vi "PathPlanner_PathPoint_Equals.vi"(9 "Other PathPlannerPoint":T1={"Position"={"X"=0.0, "Y"=0.0}, "DistAlongPath"=0.0, "MaxV"=9e+300, "Constraints"={"MaxVelocityMps;"=0.0, "MaxAccelerationMpsSq;"=0.0, "MaxAngularVelRadPsEc;"=0.0, "MaxAngularAccRadPSecSq"=0.0, "Exists"=FALSE, "Unlimited"=FALSE, "NominalVoltageVolts"=0.0}, "RotationTarget"={"rotation"={"VALUE"=0.0, "COS"=1.0, "SIN"=0.0}, "position"=1.0, "Exists"=FALSE}, "WaypointRelativePos"=0.0} {"RotationTarget"."rotation"."SIN" format="%13.4f"; "RotationTarget"."rotation"."COS" format="%13.4f"; "RotationTarget"."rotation"."VALUE" format="%13.4f"; "Position"."Y" format="%14.3f"; "Position"."X" format="%14.3f"}, 11 "PathPlannerPoint":T1={"Position"={"X"=0.0, "Y"=0.0}, "DistAlongPath"=0.0, "MaxV"=9e+300, "Constraints"={"MaxVelocityMps;"=0.0, "MaxAccelerationMpsSq;"=0.0, "MaxAngularVelRadPsEc;"=0.0, "MaxAngularAccRadPSecSq"=0.0, "Exists"=FALSE, "Unlimited"=FALSE, "NominalVoltageVolts"=0.0}, "RotationTarget"={"rotation"={"VALUE"=0.0, "COS"=1.0, "SIN"=0.0}, "position"=1.0, "Exists"=FALSE}, "WaypointRelativePos"=0.0} {"RotationTarget"."rotation"."SIN" format="%13.4f"; "RotationTarget"."rotation"."COS" format="%13.4f"; "RotationTarget"."rotation"."VALUE" format="%13.4f"; "Position"."Y" format="%14.3f"; "Position"."X" format="%14.3f"}) -> (3 "Equal":bool)   [LabVIEW 2019, in "PathPlanner24.lvlib"]
doc: "Determines if two Path Point definitions are equal\n\nInputs:\n -- PathPoint - cluster - point definition\n -- Other PathPoint - cluster - point definition\n\nOutputs:\n -- Equal - boolean - TRUE if both definitions are the same."
uses:
  PathPlanner24.lvlib
  <vilib>/Rock Robotics/WPI/ThirdParty/JAS_Junk/TrajLib/Trajectory_Library.lvlib
  <vilib>/Rock Robotics/WPI/ThirdParty/JAS_Junk/TrajLib/TypeDef/ROTATION2D.ctl
  <vilib>/Rock Robotics/WPI/ThirdParty/JAS_Junk/TrajLib/TypeDef/TRANSLATION2D.ctl
  TypeDef/PathPlannerPathConstraints.ctl
  TypeDef/PathPlannerPathPoint.ctl
  TypeDef/PathPlannerRotationTarget.ctl
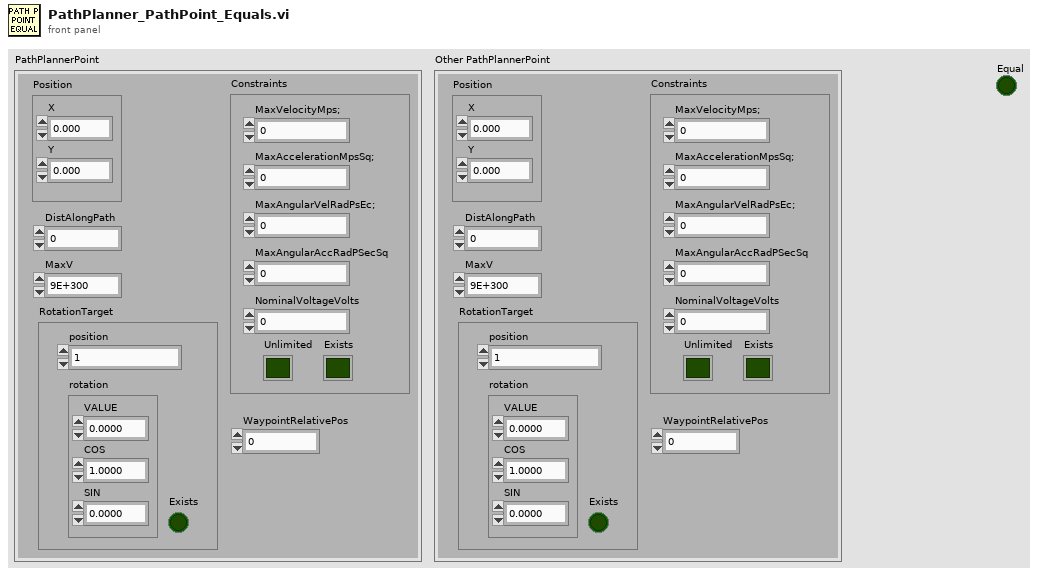
[diagram p1: front panel]
types:
  T1 = typedef "PathPlanner24.lvlib/PathPlannerPathPoint.ctl" = cluster{"Position":T2, "DistAlongPath":dbl, "MaxV":dbl, "Constraints":T3, "RotationTarget":T4, "WaypointRelativePos":dbl}
  T2 = typedef "Trajectory_Library.lvlib/TRANSLATION2D.ctl" = cluster{"X":dbl, "Y":dbl}
  T3 = typedef "PathPlanner24.lvlib/PathPlannerPathConstraints.ctl" = cluster{"MaxVelocityMps;":dbl, "MaxAccelerationMpsSq;":dbl, "MaxAngularVelRadPsEc;":dbl, "MaxAngularAccRadPSecSq":dbl, "Exists":bool, "Unlimited":bool, "NominalVoltageVolts":dbl}
  T4 = typedef "PathPlanner24.lvlib/PathPlannerRotationTarget.ctl" = cluster{"rotation":T5, "position":dbl, "Exists":bool}
  T5 = typedef "Trajectory_Library.lvlib/ROTATION2D.ctl" = cluster{"VALUE":dbl, "COS":dbl, "SIN":dbl}
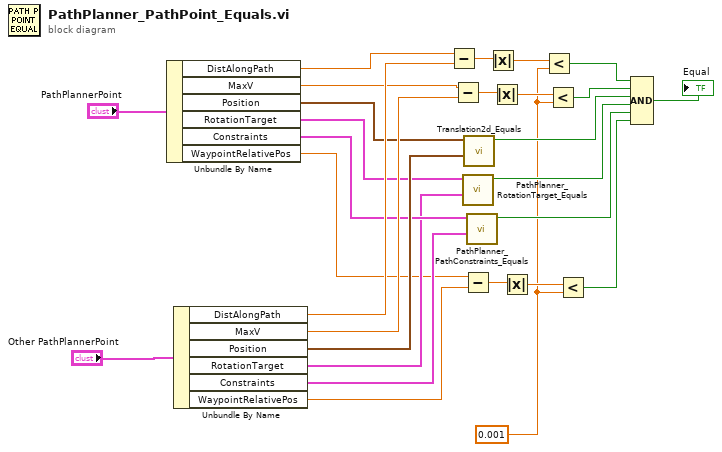
[diagram p0: block diagram]
diagram:
  w2 = 0.001 ("y")
  n1 = Unbundle By Name("PathPlannerPoint") -> ("DistAlongPath"=w26:dbl, "MaxV"=w18:dbl, "Position"=w15:T2, "RotationTarget"=w9:T4, "Constraints"=w13:T3, "WaypointRelativePos"=w4:dbl)
  n2 = Unbundle By Name("Other PathPlannerPoint") -> ("DistAlongPath"=w25:dbl, "MaxV"=w17:dbl, "Position"=w14:T2, "RotationTarget"=w8:T4, "Constraints"=w12:T3, "WaypointRelativePos"=w3:dbl)
  n3 = Subtract(x=w26, y=w25) -> (x-y=w24:dbl)
  n4 = Subtract(x=w18, y=w17) -> (x-y=w20:dbl)
  n5 = call "PathPlanner_RotationTarget_Equals.vi"("Other GoalEndState"=w8, "RotationTarget"=w9) -> ("Equal"=w7:bool)  [unwired: 9 in]
  n6 = Subtract(x=w4, y=w3) -> (x-y=w6:dbl)
  n7 = call <vilib>:"Translation2d_Equals.vi"("other Translation"=w14, "In Translation"=w15) -> ("Equals"=w11:bool)  [unwired: 9 in]
  n8 = call "PathPlanner_PathConstraints_Equals.vi"("Other PathPlannerConstraints"=w12, "PathPlannerConstraints"=w13) -> ("Equal"=w10:bool)  [unwired: 9 in]
  n9 = Absolute Value(x=w24) -> (abs(x)=w23:dbl)
  n10 = Absolute Value(x=w20) -> (abs(x)=w19:dbl)
  n11 = Absolute Value(x=w6) -> (abs(x)=w5:dbl)
  n12 = Less?(x=w23, y=w2) -> (x < y?=w22:bool)
  n13 = Less?(x=w19, y=w2) -> (x < y?=w16:bool)
  n14 = Less?(x=w5, y=w2) -> (x < y?=w1:bool)
  n15 = Compound Arithmetic op=AND(w22, w16, w11, w7, w10, w1) -> (→"Equal":bool)
